vi "OnTraceMessage.vi"(4 "TraceMessage":refnum<vi>, 5 "事件数据":cluster{"type":i32, "traceMessage":string}, 6 "控件引用":refnum<k24>, 7 "事件通用数据":cluster{"事件源":i32, "事件类型":u32, "时间标识":u32}) -> ()   [LabVIEW 2018]
uses:
  C:/users data/project/MES/MES v4.5 20250917/module/CFX/CFX_dll/CFX.dll
  CFX_dll/CFX.dll
panel:
  out "error out":errorcluster caption="错误输出"
  in  "error in":errorcluster caption="错误输入"
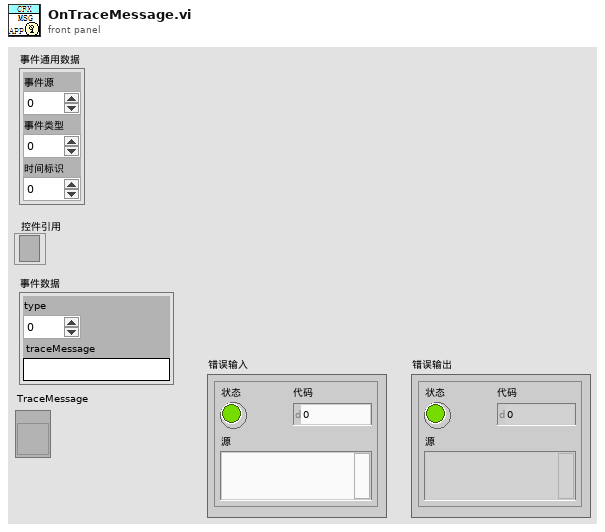
[diagram p1: front panel]
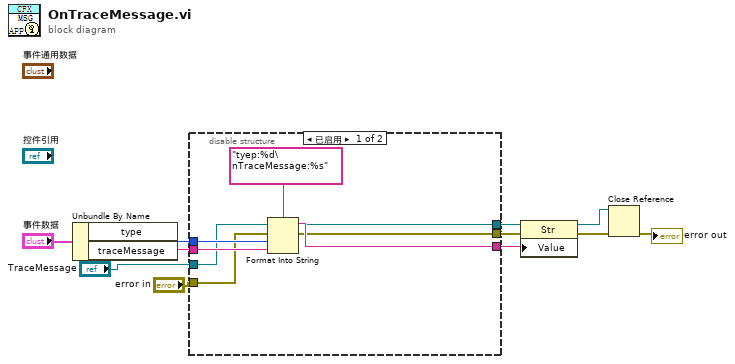
[diagram p0: block diagram]
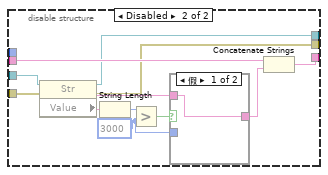
[diagram p2: hidden frame]
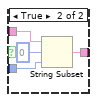
[diagram p3: hidden frame]
diagram:
  n1 = Unbundle By Name("事件数据") -> ("type"=w10:i32, "traceMessage"=w9:string)
  n2 = disable-structure shown="已启用" {
    disable-tunnel: w10 -> [w17 _]
    disable-tunnel: w9 -> [w16 w26]
    disable-tunnel: "error in" -> [w15 w20]
    disable-tunnel: [w14 w28] -> w7
    disable-tunnel: [w13 w19] -> w6
    disable-tunnel: "TraceMessage" -> [w12 w29]
    disable-tunnel: [w12 w21] -> w1
    frame Enabled {
      n3 = Format Into String(format string="tyep:%d\nTraceMessage:%s" ("格式字符串"), error in=w15, w17, w16) -> (resulting string=w14:string, error out=w13:errorcluster)  [unwired: 1 in]
    }
    frame Disabled {
      w23 = 3000 ("y")
      n4 = property class="Str"(reference=w29, error in=w20) -> (reference out=w21:refnum<vi>, error out=w19:errorcluster, "Value"=w24:string)
      n5 = String Length(string=w24) -> (length=w27:i32)
      n6 = Greater?(x=w27, y=w23) -> (0:w25:bool)
      n7 = case shown="假" w25 {
        tunnel: w24 -> [w30 w34]
        tunnel: w23 -> [_ w32]
        tunnel: [w30 w31] -> w22
        frame False {
        }
        frame True {
          n8 = String Subset(string=w34, offset (0)=0 ("偏移量(0)"), length (rest)=w32) -> (substring=w31:string)
        }
      }
      n9 = Concatenate Strings(w26, w22) -> (w28:string)
    }
  }
  n10 = property class="Str"(reference=w1, error in=w6, "Value"=w7) -> (reference out=w4:refnum<vi>, error out=w3:errorcluster)
  n11 = Close Reference(reference=w4, error in (no error)=w3) -> (error out=→"error out":errorcluster)
